vi "Start Streamed Request.vi"(0 "stream?":bool, 1 "id in":i32, 2 "protocol version":string, 3 "Mcp-Method":string, 5 "events":refnum<queue>, 7 "cancelled":refnum<queue>, 9 "request":string, 11 "error in":errorcluster, 12 "Mcp-Name":string) -> (15 "error out":errorcluster)   [LabVIEW 2020, in "MCP Server.lvlib"]
doc: "When stream? is TRUE, starts Run Streamed Request.vi (same folder) in the background for one streamed tools/call and returns at once, so that Process HTTP Request.vi can hand the MCP SSE Response to the IG HTTP Server, which then sends each event as it is queued. The VI is opened as a reentrant clone (Open VI Reference option 0x08), its controls are set by name and it is run with Wait until done FALSE and Auto Dispose Ref TRUE: fire and forget.\n\nWhen stream? is FALSE the two queues are released (Process HTTP Request.vi creates the MCP SSE Response for every request). When the start fails, the end marker is queued so that the stream ends instead of waiting forever, and the error is returned."
uses:
  MCP Server.lvlib
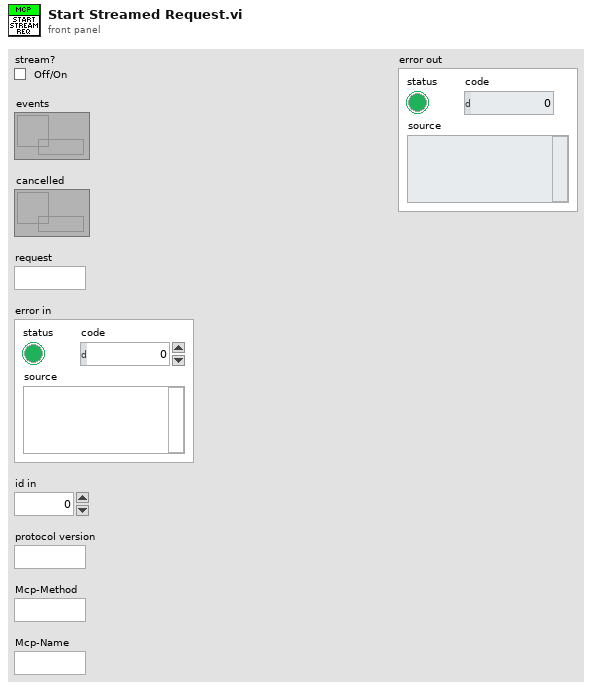
[diagram p1: front panel]
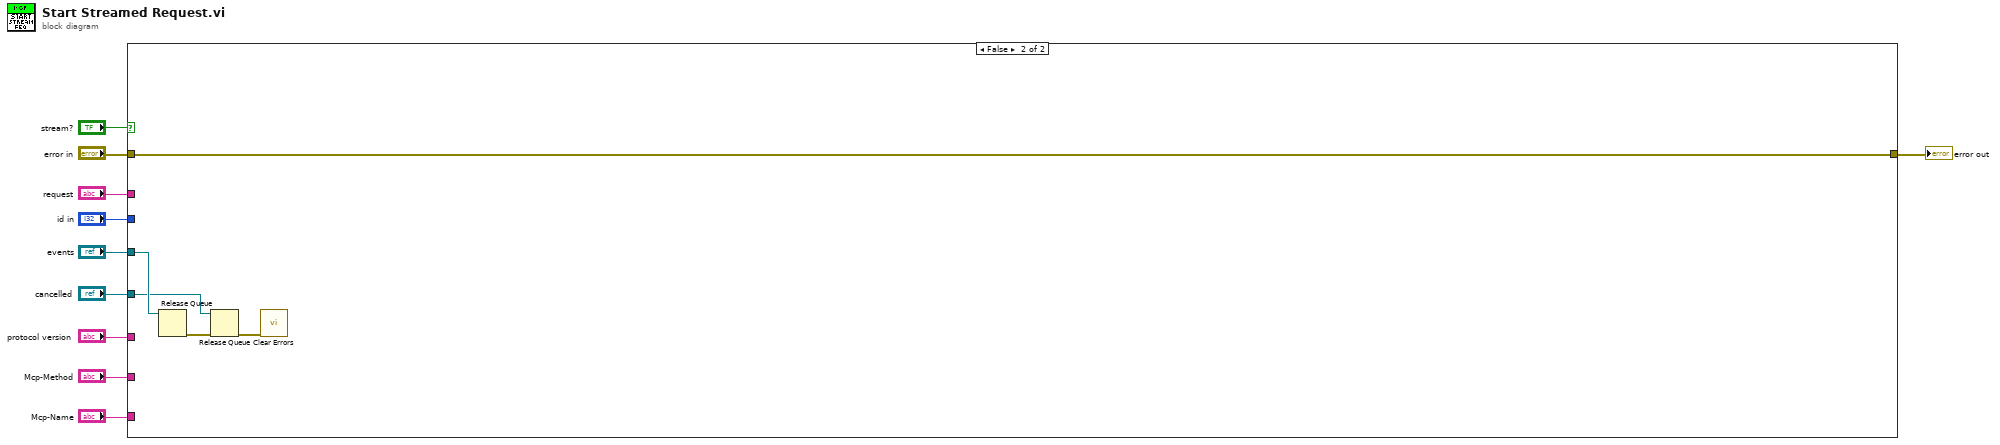
[diagram p0: block diagram]
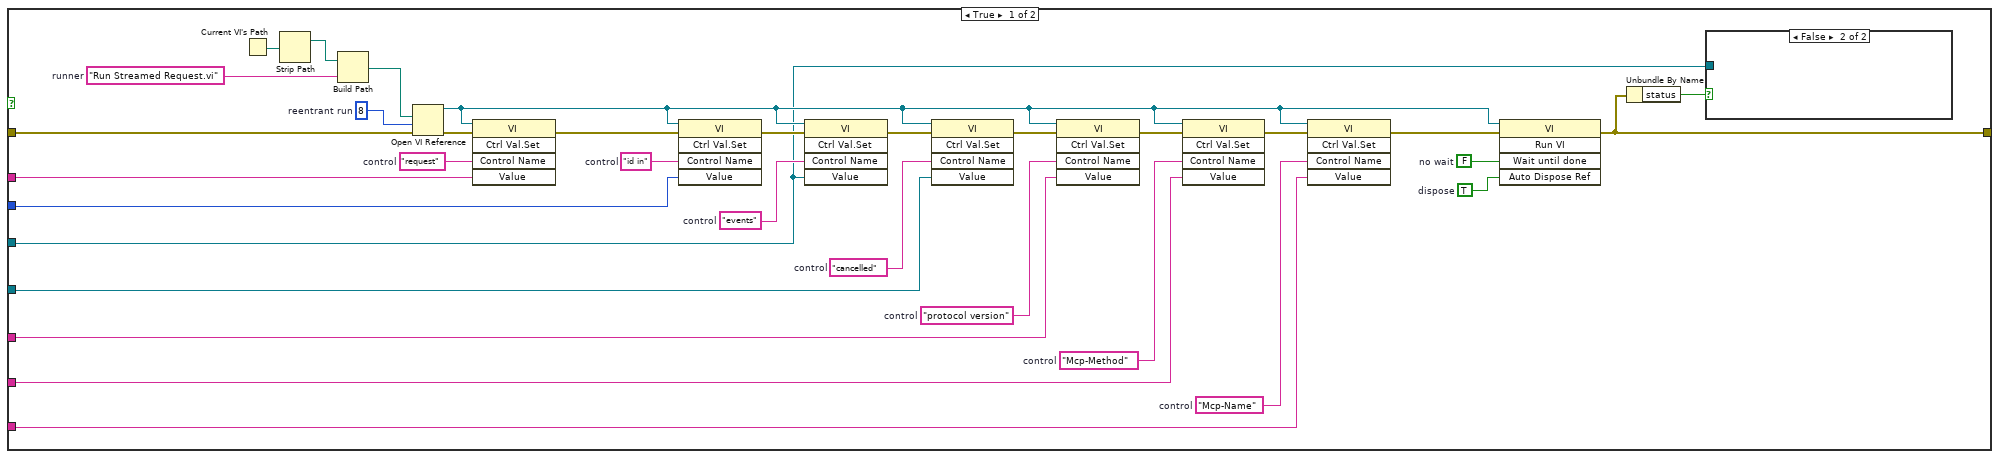
[diagram p2: hidden frame]
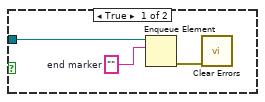
[diagram p3: hidden frame]
diagram:
  n1 = case shown="False" "stream?" {
    tunnel: "events" -> [w13 w51]
    tunnel: "cancelled" -> [w27 w50]
    tunnel: "request" -> [w35 _]
    tunnel: "id in" -> [w32 _]
    tunnel: "protocol version" -> [w24 _]
    tunnel: "Mcp-Method" -> [w21 _]
    tunnel: "Mcp-Name" -> [w18 _]
    tunnel: "error in" -> [w38 w47]
    tunnel: [w11 w47] -> w1
    frame True {
      w14 = TRUE  # dispose
      w15 = FALSE  # no wait
      w19 = "Mcp-Name"  # control
      w22 = "Mcp-Method"  # control
      w25 = "protocol version"  # control
      w28 = "cancelled"  # control
      w30 = "events"  # control
      w33 = "id in"  # control
      w36 = "request"  # control
      w39 = u32 8  # reentrant run
      w41 = "Run Streamed Request.vi"  # runner
      n2 = Current VI's Path() -> (path=w43:path)
      n3 = Strip Path(path=w43) -> (stripped path=w42:path)  [unwired: 1 out]
      n4 = Build Path(base path=w42, name or relative path=w41) -> (appended path=w40:path)
      n5 = Open VI Reference(vi path=w40, options=w39, error in (no error)=w38) -> (vi reference=w17:refnum<vi>, error out=w37:errorcluster)  [unwired: 3 in]
      n6 = invoke class="VI" method="Ctrl Val.Set"(reference=w17, error in=w37, "Control Name"=w36, "Value"=w35) -> (error out=w34:errorcluster)  [unwired: 1 in, 4 out]
      n7 = invoke class="VI" method="Ctrl Val.Set"(reference=w17, error in=w34, "Control Name"=w33, "Value"=w32) -> (error out=w31:errorcluster)  [unwired: 1 in, 4 out]
      n8 = invoke class="VI" method="Ctrl Val.Set"(reference=w17, error in=w31, "Control Name"=w30, "Value"=w13) -> (error out=w29:errorcluster)  [unwired: 1 in, 4 out]
      n9 = invoke class="VI" method="Ctrl Val.Set"(reference=w17, error in=w29, "Control Name"=w28, "Value"=w27) -> (error out=w26:errorcluster)  [unwired: 1 in, 4 out]
      n10 = invoke class="VI" method="Ctrl Val.Set"(reference=w17, error in=w26, "Control Name"=w25, "Value"=w24) -> (error out=w23:errorcluster)  [unwired: 1 in, 4 out]
      n11 = invoke class="VI" method="Ctrl Val.Set"(reference=w17, error in=w23, "Control Name"=w22, "Value"=w21) -> (error out=w20:errorcluster)  [unwired: 1 in, 4 out]
      n12 = invoke class="VI" method="Ctrl Val.Set"(reference=w17, error in=w20, "Control Name"=w19, "Value"=w18) -> (error out=w16:errorcluster)  [unwired: 1 in, 4 out]
      n13 = invoke class="VI" method="Run VI"(reference=w17, error in=w16, "Wait until done"=w15, "Auto Dispose Ref"=w14) -> (error out=w11:errorcluster)  [unwired: 1 in, 4 out]
      n14 = Unbundle By Name(w11) -> ("status"=w12:bool)
      n15 = case shown="False" w12 {
        tunnel: w13 -> [w46 _]
        frame True {
          w45 = ""  # end marker
          n16 = Enqueue Element(queue=w46, element=w45) -> (error out=w44:errorcluster)  [unwired: 2 in, 2 out]
          n17 = call <vilib>:"Clear Errors.vi"("error in (no error)"=w44) -> ()  [unwired: 5 in, 2 out]
        }
        frame False {
        }
      }
    }
    frame False {
      n18 = Release Queue(queue=w51) -> (error out=w49:errorcluster)  [unwired: 2 in, 2 out]
      n19 = Release Queue(queue=w50, error in (no error)=w49) -> (error out=w48:errorcluster)  [unwired: 1 in, 2 out]
      n20 = call <vilib>:"Clear Errors.vi"("error in (no error)"=w48) -> ()  [unwired: 5 in, 2 out]
    }
  }
  "error out" <- w1
